vi "WritePara.vi"(0 "TRIG_TH":i32=200, 1 "error in":errorcluster, 2 "BL_LEN":i32=50, 3 "EVT_LEN":i32=400, 4 "TRIG_DL":i32=500, 5 "BPM:DIA":i32=50, 6 "TRIG_DT":i32=500, 7 "EVT_TAIL":i32=300, 9 "connection ID in":refnum<k5>) -> (8 "error out":errorcluster)   [LabVIEW 2014]
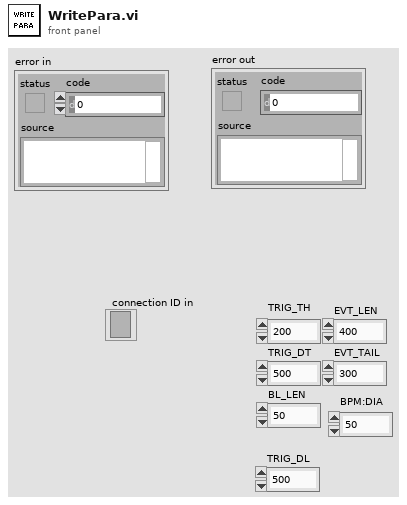
[diagram p1: front panel]
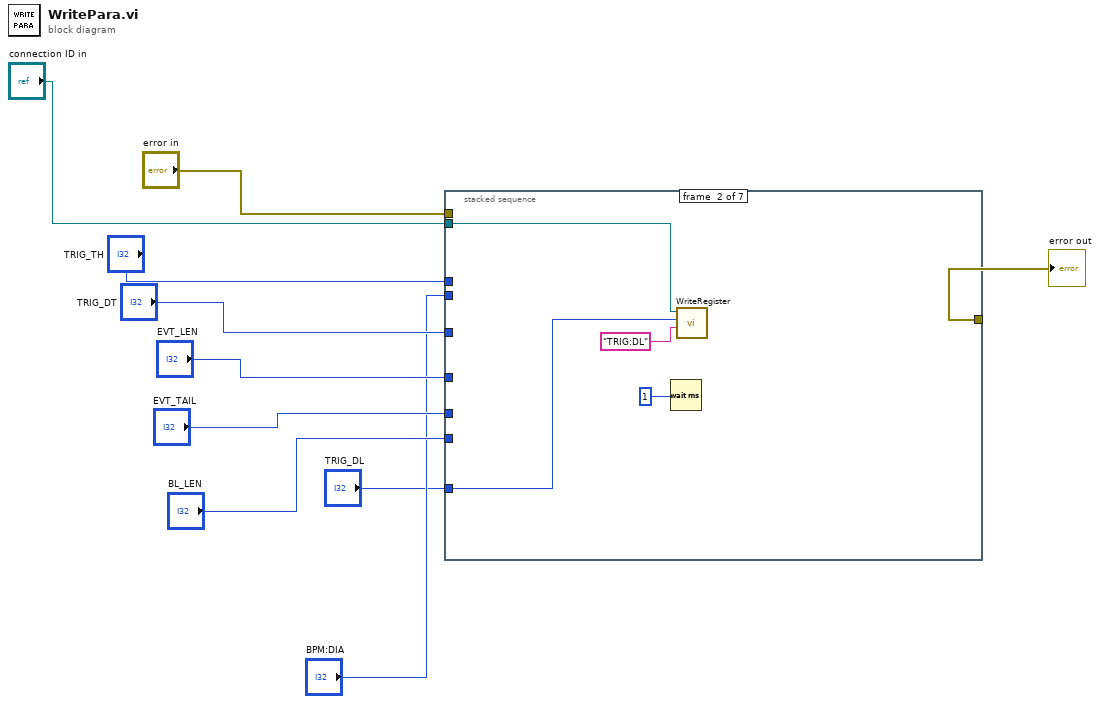
[diagram p0: block diagram]
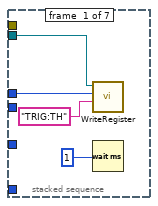
[diagram p2: hidden frame]
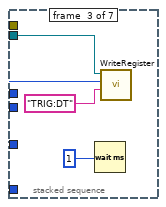
[diagram p3: hidden frame]
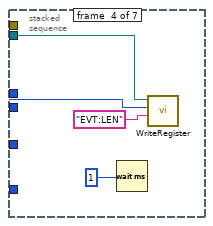
[diagram p4: hidden frame]
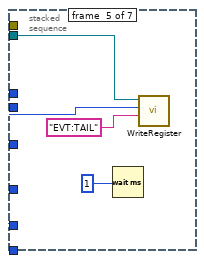
[diagram p5: hidden frame]
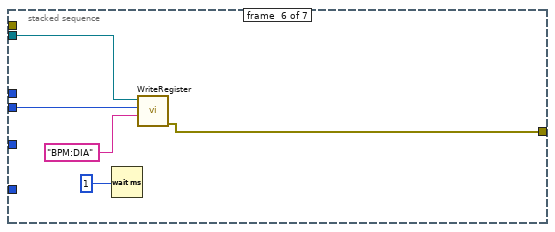
[diagram p6: hidden frame]
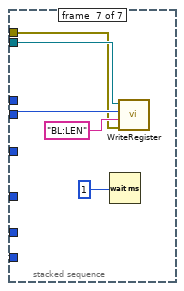
[diagram p7: hidden frame]
diagram:
  n1 = stacked-sequence {
    tunnel: "TRIG_TH" -> [w12 _ _ _ _ _ _]
    tunnel: "connection ID in" -> [w11 w15 w19 w24 w28 w34 w38]
    tunnel: "TRIG_DT" -> [_ _ w20 _ _ _ _]
    tunnel: "EVT_LEN" -> [_ _ _ w23 _ _ _]
    tunnel: "EVT_TAIL" -> [_ _ _ _ w29 _ _]
    tunnel: "BL_LEN" -> [_ _ _ _ _ _ w39]
    tunnel: [_ _ _ _ _ w31 _] -> w4
    tunnel: "error in" -> [_ _ _ _ _ _ w36]
    tunnel: "BPM:DIA" -> [_ _ _ _ _ w32 _]
    tunnel: "TRIG_DL" -> [_ w16 _ _ _ _ _]
    frame #0 {
      n2 = call "WriteRegister.vi"("string in"="TRIG:TH", "value in"=w12, "connection ID in"=w11) -> ()  [unwired: 5 in, 2 out]
      n3 = Wait (ms)(milliseconds to wait=1 ("Value")) -> ()  [unwired: 1 out]
    }
    frame #1 {
      n4 = Wait (ms)(milliseconds to wait=1 ("Value")) -> ()  [unwired: 1 out]
      n5 = call "WriteRegister.vi"("string in"="TRIG:DL", "value in"=w16, "connection ID in"=w15) -> ()  [unwired: 5 in, 2 out]
    }
    frame #2 {
      n6 = Wait (ms)(milliseconds to wait=1 ("Value")) -> ()  [unwired: 1 out]
      n7 = call "WriteRegister.vi"("string in"="TRIG:DT", "value in"=w20, "connection ID in"=w19) -> ()  [unwired: 5 in, 2 out]
    }
    frame #3 {
      n8 = Wait (ms)(milliseconds to wait=1 ("Value")) -> ()  [unwired: 1 out]
      n9 = call "WriteRegister.vi"("string in"="EVT:LEN", "value in"=w23, "connection ID in"=w24) -> ()  [unwired: 5 in, 2 out]
    }
    frame #4 {
      n10 = Wait (ms)(milliseconds to wait=1 ("Value")) -> ()  [unwired: 1 out]
      n11 = call "WriteRegister.vi"("string in"="EVT:TAIL", "value in"=w29, "connection ID in"=w28) -> ()  [unwired: 5 in, 2 out]
    }
    frame #5 {
      n12 = Wait (ms)(milliseconds to wait=1 ("Value")) -> ()  [unwired: 1 out]
      n13 = call "WriteRegister.vi"("string in"="BPM:DIA", "value in"=w32, "connection ID in"=w34) -> ("error out"=w31:errorcluster)  [unwired: 5 in, 1 out]
    }
    frame #6 {
      n14 = Wait (ms)(milliseconds to wait=1 ("Value")) -> ()  [unwired: 1 out]
      n15 = call "WriteRegister.vi"("error in"=w36, "string in"="BL:LEN", "value in"=w39, "connection ID in"=w38) -> ()  [unwired: 4 in, 2 out]
    }
  }
  "error out" <- w4
